vi "Synth_Ending_Frequency.vi"(11 "Ending Frequency":string) -> ()   [LabVIEW 2024]
uses:
  Serial Port.vi
  <vilib>/Instr/_visa.llb/VISA Configure Serial Port (Instr).vi
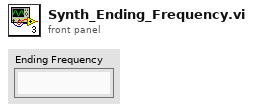
[diagram p1: front panel]
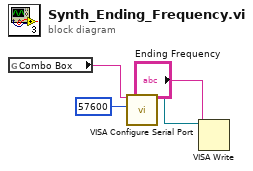
[diagram p0: block diagram]
diagram:
  n1 = global read "Serial Port.vi" "Combo Box"() -> (w1:string)
  n2 = call-poly "VISA Configure Serial Port"("VISA resource name"=w1, "baud rate (9600)"=u32 57600) -> ("VISA resource name out"=w3:refnum<visa-resource-name>)  [unwired: 12 in, 1 out]
  n3 = VISA Write(VISA resource name=w3, write buffer="Ending Frequency") -> ()  [unwired: 1 in, 3 out]
